vi "MQTT Session - Get Data.vi"(0 "mqtt ref in":T1, 11 "error in":errorcluster) -> (4 "mqtt ref out":T1, 8 "mqtt ref data":T2={"TCP ref"=refnum, "Next Packet Id"=0, "Version"=0, "Host"="localhost", "Port"=1883, "Ping Delta"=60, "Username"="", "Password"="", "Will QoS"=0, "Will Retain"=FALSE, "Will Topic"="", "Will Payload"="", "TCP Timeout"=1000, "Semaphore"=refnum, "In-Flight Messages"=variant, "Close"=FALSE, "Last Send"=0, "Keep Alive"=0, "Last Ping RTT"=0, "Last Ping"=0, "Will Properties"=[], "Session Expiry Interval"=0, "Maximum QoS"=0, "Retain Available"=FALSE, "Server Maximum Packet Size"=0, "Client Identifier"="", "Server Topic Alias Maximum"=0, "Wildcard Subscription Available"=FALSE, "Subscription Identifier Available"=FALSE, "Shared Subscription Available"=FALSE, "Connect Properties"=[], "Client Maximum Packet Size"=0, "Client Topic Alias Maximum"=0, "Server Receive Maximum"=0, "Client Receive Maximum"=0, "TLS cfg"=refnum, "Subscriptions"=[]} {"Connect Properties"."Property" items=[" Session Expiry Interval           "=17, " Authentication Method             "=21, " Authentication Data               "=22, " Request Problem Information       "=23, " Request Response Information      "=25, " Receive Maximum                   "=33, " Topic Alias Maximum               "=34, " User Property                     "=38, " Maximum Packet Size               "=39]; "Will Properties"."Property" items=[" Payload Format Indicator          "=1, " Message Expiry Interval           "=2, " Content Type                      "=3, " Response Topic                    "=8, " Correlation Data                  "=9, " Will Delay Interval               "=24, " User Property                     "=38]}, 15 "error out":errorcluster)   [LabVIEW 2019, in "KoRE-MQTT.lvlib"]
doc: "Copyright (c) 2025 KoRElibs.com\nSPDX-License-Identifier: EUPL-1.2\n\nThis VI is licensed under the European Union Public License (EUPL) Version 1.2. You may use this VI unmodified in proprietary works. If you distribute a modified version of this file, the modified file must be released under the EUPL-1.2. Full license: https://joinup.ec.europa.eu/asset/eupl/eupl/1.2/"
uses:
  KoRE-MQTT.lvlib
  Public/TypeDefs/MQTT Client Session - Data.ctl
  Public/TypeDefs/MQTT Property - Will.ctl
  Public/TypeDefs/MQTT Property - CONNECT.ctl
  TypeDefs/MQTT Subscription - Info.ctl
  Public/TypeDefs/MQTT Client Session.ctl
  TypeDefs/MQTT Client Session - Data Value Reference.ctl
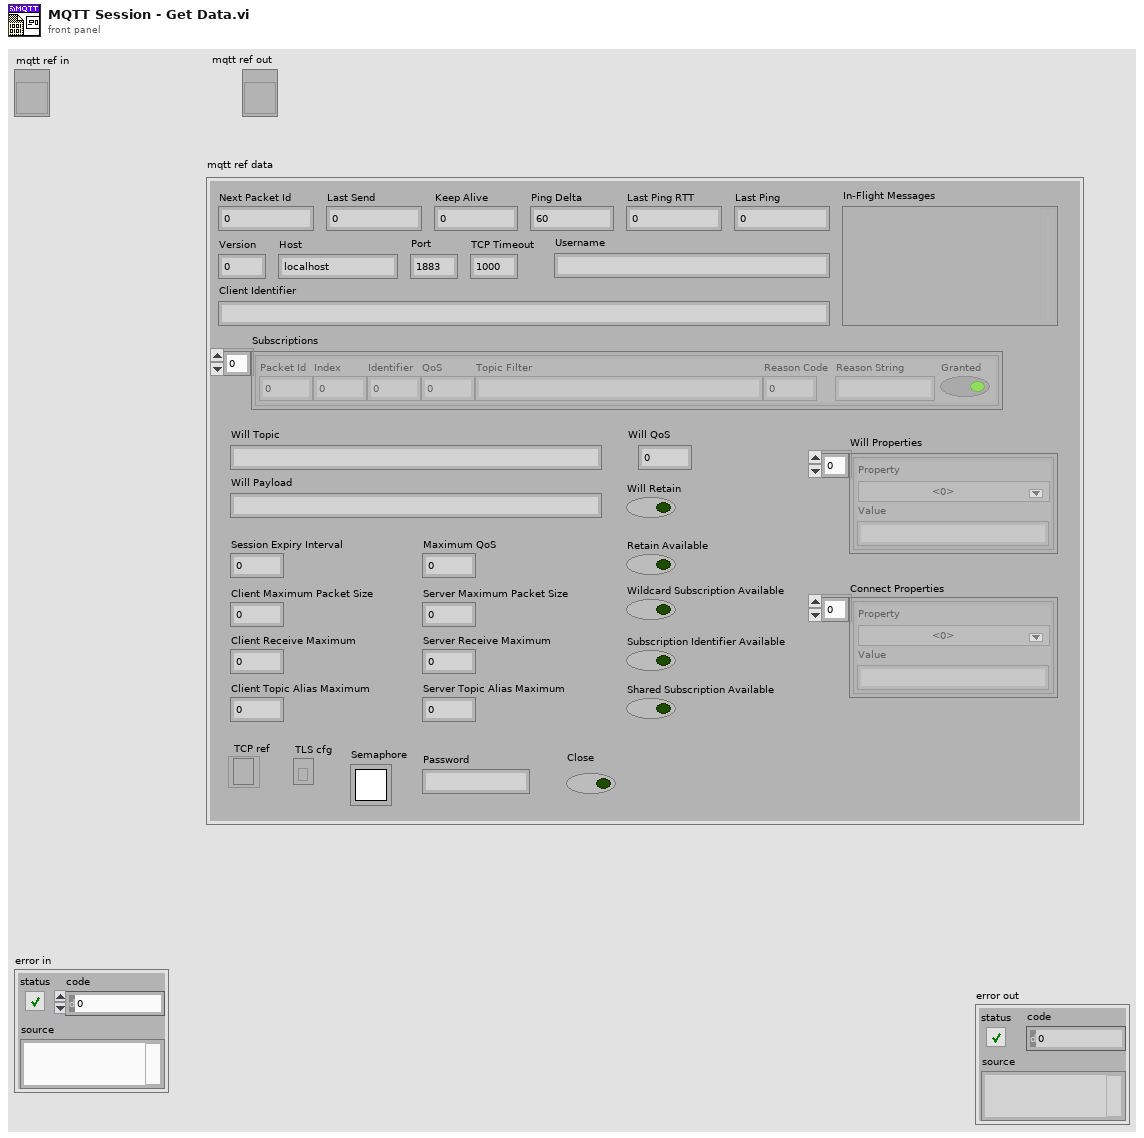
[diagram p1: front panel]
types:
  T1 = typedef "KoRE-MQTT.lvlib/MQTT Client Session.ctl" = refnum<vi>
  T2 = typedef "KoRE-MQTT.lvlib/MQTT Client Session - Data.ctl" = cluster{"TCP ref":refnum<k5>, "Next Packet Id":u16, "Version":u8, "Host":string, "Port":u16, "Ping Delta":u32, "Username":string, "Password":string, "Will QoS":u8, "Will Retain":bool, "Will Topic":string, "Will Payload":string, "TCP Timeout":i32, "Semaphore":T3, "In-Flight Messages":variant, "Close":bool, "Last Send":u32, "Keep Alive":u16, "Last Ping RTT":u32, "Last Ping":u32, "Will Properties":T4[], "Session Expiry Interval":u32, "Maximum QoS":u8, "Retain Available":bool, "Server Maximum Packet Size":u32, "Client Identifier":string, "Server Topic Alias Maximum":u16, "Wildcard Subscription Available":bool, "Subscription Identifier Available":bool, "Shared Subscription Available":bool, "Connect Properties":T5[], "Client Maximum Packet Size":u32, "Client Topic Alias Maximum":u16, "Server Receive Maximum":u16, "Client Receive Maximum":u16, "TLS cfg":refnum<k36>, "Subscriptions":T6[]}
  T3 = typedef "Semaphore RefNum" = refnum<k1>
  T4 = typedef "KoRE-MQTT.lvlib/MQTT Property - Will.ctl" = cluster{"Property":u8, "Value":string}
  T5 = typedef "KoRE-MQTT.lvlib/MQTT Property - CONNECT.ctl" = cluster{"Property":u8, "Value":string}
  T6 = typedef "KoRE-MQTT.lvlib/MQTT Subscription - Info.ctl" = cluster{"Packet Id":u16, "Index":u16, "Identifier":u32, "QoS":u8, "Topic Filter":string, "Reason Code":u8, "Reason String":string, "Granted":bool}
  T7 = typedef "KoRE-MQTT.lvlib/MQTT Client Session - Data Value Reference.ctl" = refnum<data-value>
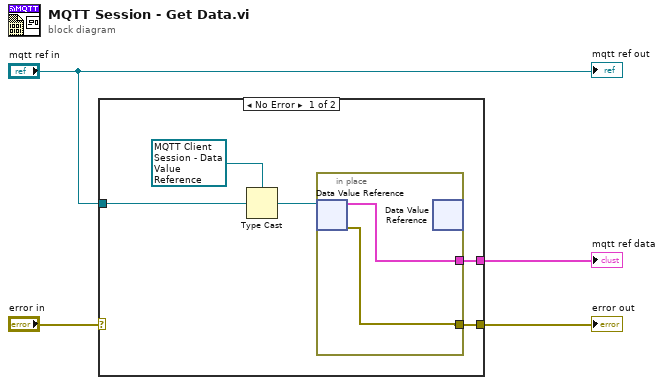
[diagram p0: block diagram]
diagram:
  n1 = case shown="No Error" "error in" {
    selector: "error in" -> [_ w12]
    tunnel: "mqtt ref in" -> [w7 _]
    tunnel: [w6 w12] -> w3
    tunnel: [w5 _] -> w1
    frame No Error {
      n2 = Type Cast(type=T7 refnum ("data value reference"), x=w7) -> (*(type *) &x=w8:T7)
      n3 = in-place "In Place Element Structure" {
        in-place-border: [w11] -> w5
        in-place-border: [w10] -> w6
        n4 = in-place-dvr #1(w8) -> (w11:T2, w10:errorcluster)
        n5 = in-place-dvr #1() -> ()  [unwired: 1 in, 2 out]
      }
    }
    frame Error {
    }
  }
  "error out" <- w3
  "mqtt ref data" <- w1
  "mqtt ref out" <- "mqtt ref in"
